vi "Display Probe NI.vi"(0 "x":dbl) -> (4 "negative?":bool, 6 "joined":string, 8 "array":dbl[](array[numeric]))   [LabVIEW 2026]
doc: "Probe: constant labels, whitespace string, array constant, error constant, loop stop terminal, comparison with zero."
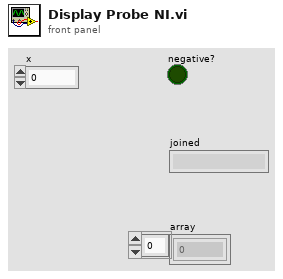
[diagram p1: front panel]
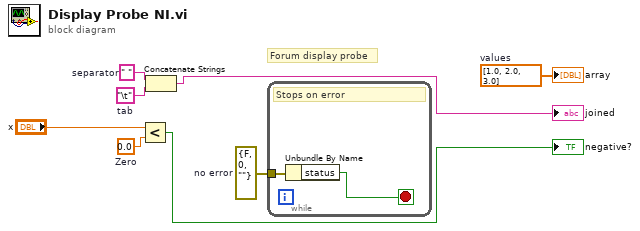
[diagram p0: block diagram]
diagram:
  w1 = errorcluster {"status"=FALSE, "code"=0, "source"=""}  # no error
  w2 = dbl[] [1.0, 2.0, 3.0]  # values
  w4 = "\t"  # tab
  w5 = " "  # separator
  w7 = 0.0  # Zero
  # "Forum display probe"
  n1 = Less?(x="x", y=w7) -> (x < y?=→"negative?":bool)
  n2 = Concatenate Strings(w5, w4) -> (→"joined":string)
  n3 = while {
    tunnel: w1 -> [w10]
    stop <- w9 stop-if-true
    # "Stops on error"
    n4 = Unbundle By Name(w10) -> ("status"=w9:bool)
  }
  "array" <- w2
